vi "Create Constructor.vi"(8 "error in (no error)":errorcluster, 11 "Mock Class Generator in":refnum<class "Mock Class Generator.lvclass">) -> (0 "error out":errorcluster, 2 "Created Constructor":path[](array[path]), 3 "Mock Class Generator":refnum<class "Mock Class Generator.lvclass">)   [LabVIEW 2020, in "Mock Class Generator.lvclass"]
uses:
  Mock Class Generator.lvclass
  Mock Class Generator.lvclass/Mock Class Generator.ctl
  Templates/Create.vi
  Templates/Templates.lvlib
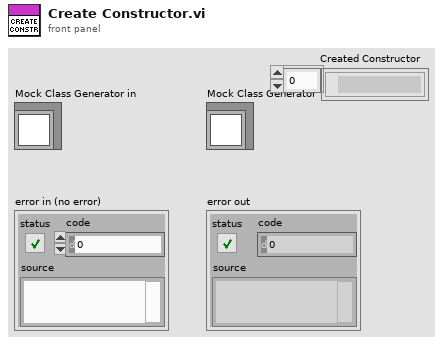
[diagram p1: front panel]
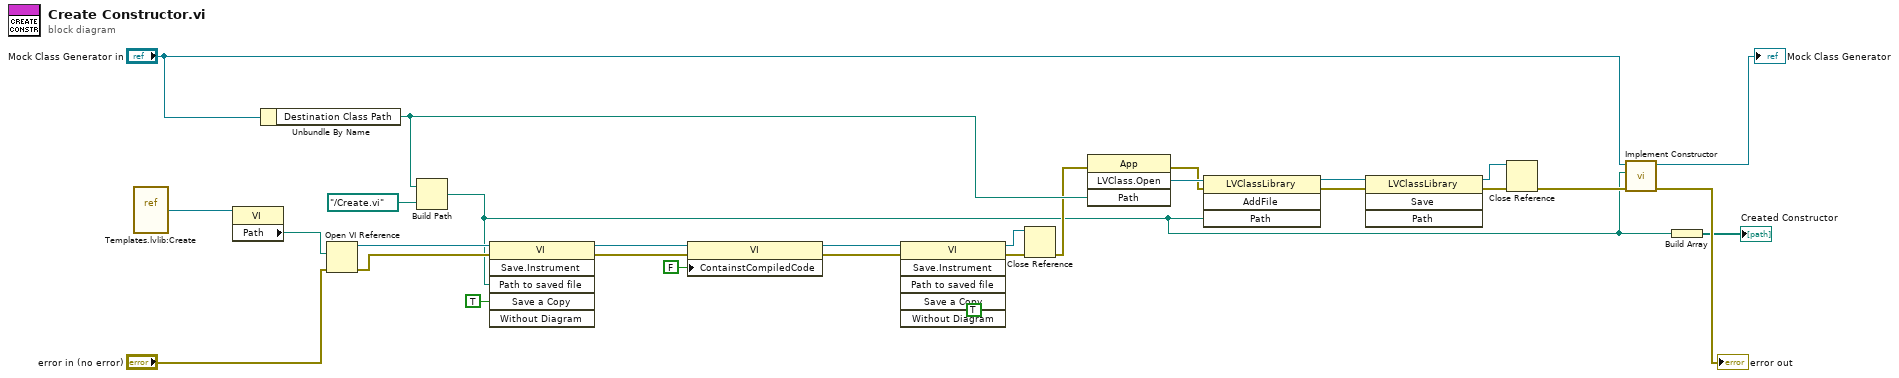
[diagram p0: block diagram]
diagram:
  (unwired) TRUE ("Save a Copy")
  n1 = vi-ref "Templates.lvlib:Create.vi"() -> (w17:refnum<vi>)
  n2 = property class="VI"(reference=w17) -> ("Path"=w16:path)  [unwired: 1 in, 2 out]
  n3 = Unbundle By Name("Mock Class Generator in") -> ("Destination Class Path"=w25:path)
  n4 = Open VI Reference(vi path=w16, error in (no error)="error in (no error)") -> (vi reference=w4:refnum<vi>, error out=w15:errorcluster)  [unwired: 4 in]
  n5 = Build Path(base path=w25, name or relative path=path "../Create.vi") -> (appended path=w2:path)
  n6 = invoke class="VI" method="Save.Instrument"(reference=w4, error in=w15, "Path to saved file"=w2, "Save a Copy"=TRUE) -> (reference out=w3:refnum<vi>, error out=w5:errorcluster)  [unwired: 2 in, 4 out]
  n7 = property class="VI"(reference=w3, error in=w5, "ContainstCompiledCode"=FALSE ("Contains Compiled Code")) -> (reference out=w7:refnum<vi>, error out=w8:errorcluster)
  n8 = invoke class="VI" method="Save.Instrument"(reference=w7, error in=w8) -> (reference out=w23:refnum<vi>, error out=w26:errorcluster)  [unwired: 4 in, 4 out]
  n9 = Close Reference(reference=w23, error in (no error)=w26) -> (error out=w22:errorcluster)
  n10 = invoke class="App" method="LVClass.Open"(error in=w22, "Path"=w25) -> (error out=w21:errorcluster, "LVClass.Open"=w28:refnum<vi>)  [unwired: 2 in, 2 out]
  n11 = invoke class="LVClassLibrary" method="AddFile"(reference=w28, error in=w21, "Path"=w2) -> (reference out=w20:refnum<vi>, error out=w19:errorcluster)  [unwired: 1 in, 2 out]
  n12 = invoke class="LVClassLibrary" method="Save"(reference=w20, error in=w19) -> (reference out=w13:refnum<vi>, error out=w18:errorcluster)  [unwired: 2 in, 2 out]
  n13 = Close Reference(reference=w13, error in (no error)=w18) -> (error out=w12:errorcluster)
  n14 = call "Implement Constructor.vi"("error in (no error)"=w12, "Constructor Path"=w2, "Mock Class Generator in"="Mock Class Generator in") -> ("error out"=→"error out":errorcluster, "Mock Class Generator"=→"Mock Class Generator":refnum<class "Mock Class Generator.lvclass">)  [unwired: 7 in]
  n15 = Build Array(w2) -> (→"Created Constructor":path[])
